vi "Build Status.vi"(11 "Git Info":T2) -> (0 "Remote Color":u32(colorbox)=13816530, 1 "Remote Status":string, 2 "Local Color":u32(colorbox)=13816530, 3 "Local Status":string, 4 "Commit":T1(ring), 5 "Revert":T1(ring), 6 "Pull":T1(ring), 8 "Push":T1(ring))   [LabVIEW 2020, in "VolatusGUI.lvlib" / "Git Updater Module.lvclass"]
uses:
  Git Updater Module.lvclass
  Git Info.ctl
  <vilib>/Hampel Software Engineering/Git API/Git API/Controls/GIT-Repository States.ctl
  <vilib>/Hampel Software Engineering/Git API/Git API/GIT-api.lvclass
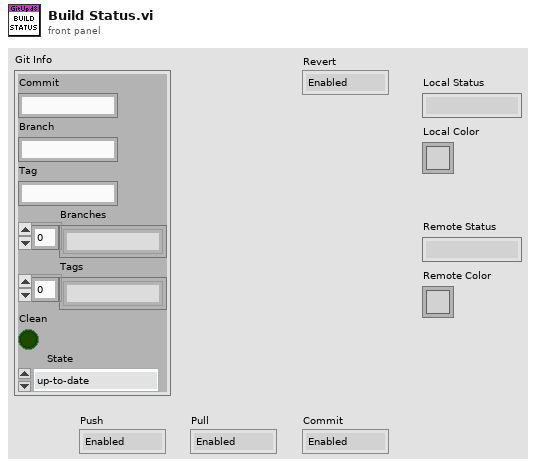
[diagram p1: front panel]
types:
  T1 = enum8{"Enabled", "Disabled", "Disabled and Grayed Out"}
  T2 = typedef "VolatusGUI.lvlib/Git Updater Module.lvclass/Git Info.ctl" = cluster{"Commit":string, "Branch":string, "Tag":string, "Branches":string[], "Tags":string[], "Clean":bool, "State":T3}
  T3 = typedef "GIT-API-for-LabVIEW.lvlib/GIT-api.lvclass/GIT-Repository States.ctl" = enum16{"up-to-date", "behind", "ahead", "diverged", "unpublished", "detached", "unknown"}
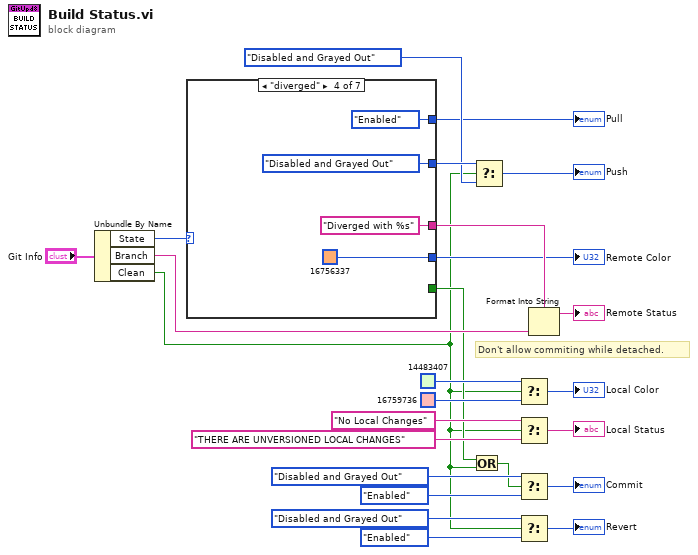
[diagram p0: block diagram]
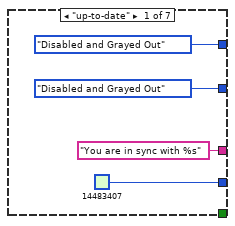
[diagram p2: hidden frame]
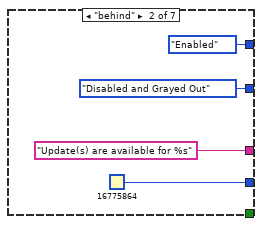
[diagram p3: hidden frame]
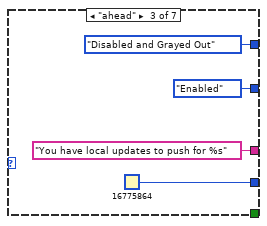
[diagram p4: hidden frame]
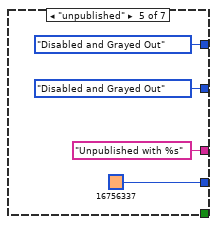
[diagram p5: hidden frame]
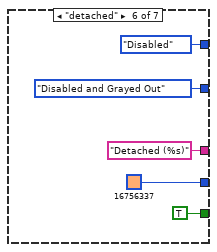
[diagram p6: hidden frame]
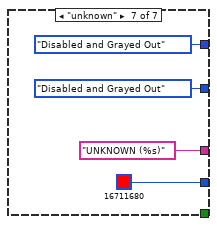
[diagram p7: hidden frame]
diagram:
  # "Don't allow commiting while detached."
  n1 = Unbundle By Name("Git Info") -> ("State"=w24:T3, "Branch"=w22:string, "Clean"=w3:bool)
  n2 = case shown="\"diverged\"" w24 {
    tunnel: ["You are in sync with %s" "Update(s) are available for %s" "You have local updates to push for %s" "Diverged with %s" "Unpublished with %s" "Detached (%s)" "UNKNOWN (%s)"] -> w23
    tunnel: [u32 14483407 u32 16775864 u32 16775864 u32 16756337 u32 16756337 u32 16756337 u32 16711680] -> w18
    tunnel: [T1."Disabled and Grayed Out" ("Commit") T1."Enabled" ("Commit") T1."Disabled and Grayed Out" ("Commit") T1."Enabled" ("Commit") T1."Disabled and Grayed Out" ("Commit") T1."Disabled" ("Commit") T1."Disabled and Grayed Out" ("Commit")] -> w1
    tunnel: [T1."Disabled and Grayed Out" ("Commit") T1."Disabled and Grayed Out" ("Commit") T1."Enabled" ("Commit") T1."Disabled and Grayed Out" ("Commit") T1."Disabled and Grayed Out" ("Commit") T1."Disabled and Grayed Out" ("Commit") T1."Disabled and Grayed Out" ("Commit")] -> w10
    tunnel: [_ _ _ _ _ TRUE _] -> w6
    frame "up-to-date" {
    }
    frame "behind" {
    }
    frame "ahead" {
    }
    frame "diverged" {
    }
    frame "unpublished" {
    }
    frame "detached" {
    }
    frame "unknown" {
    }
  }
  "Remote Color" <- w18
  "Pull" <- w1
  n3 = Or(x=w6, y=w3) -> (x .or. y?=w7:bool)
  n4 = Select(t=w10, s=w3, f=T1."Disabled and Grayed Out" ("Commit")) -> (s? t:f=→"Push":T1)
  n5 = Select(t=u32 14483407, s=w3, f=u32 16759736) -> (s? t:f=→"Local Color":u32)
  n6 = Select(t="No Local Changes", s=w3, f="THERE ARE UNVERSIONED LOCAL CHANGES") -> (s? t:f=→"Local Status":string)
  n7 = Select(t=T1."Disabled and Grayed Out" ("Commit"), s=w7, f=T1."Enabled" ("Commit")) -> (s? t:f=→"Commit":T1)
  n8 = Select(t=T1."Disabled and Grayed Out" ("Commit"), s=w3, f=T1."Enabled" ("Commit")) -> (s? t:f=→"Revert":T1)
  n9 = Format Into String(format string=w23, w22) -> (resulting string=→"Remote Status":string)  [unwired: 2 in, 1 out]
